vi "Log File Name for Mode.vi"(8 "error in":errorcluster, 9 "Mode":T1, 10 "base path":path) -> (0 "error out":errorcluster, 1 "for input Mode":path, 2 "for Create New":path, 3 "for Append":path, 5 "for Overwrite":path)   [LabVIEW 2021, in "Logging.lvlib"]
doc: "Take 'base path' and format it for presentation in the UI."
uses:
  Logging.lvlib
  Logging Mode.ctl
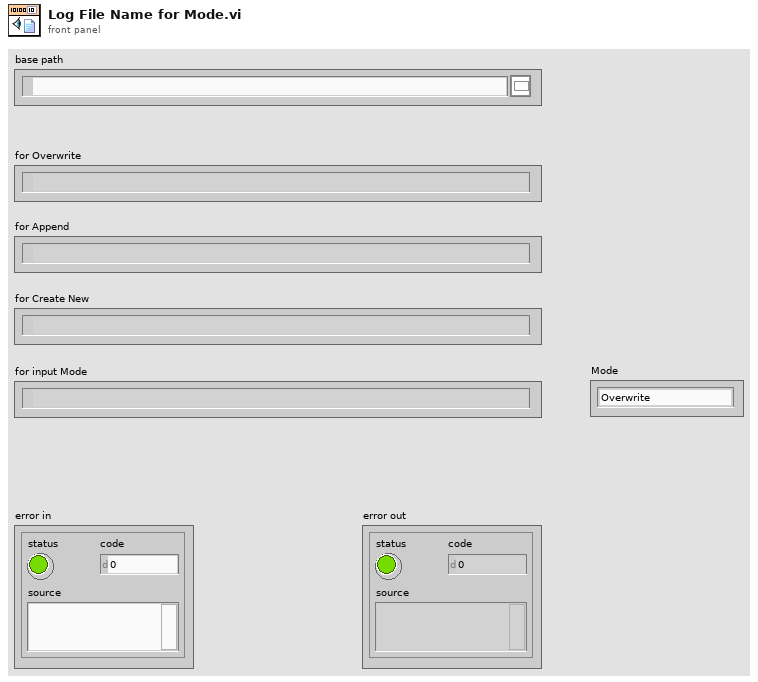
[diagram p1: front panel]
types:
  T1 = typedef "Logging.lvlib/Logging Mode.ctl" = enum16{"Overwrite", "Append", "Create New"}
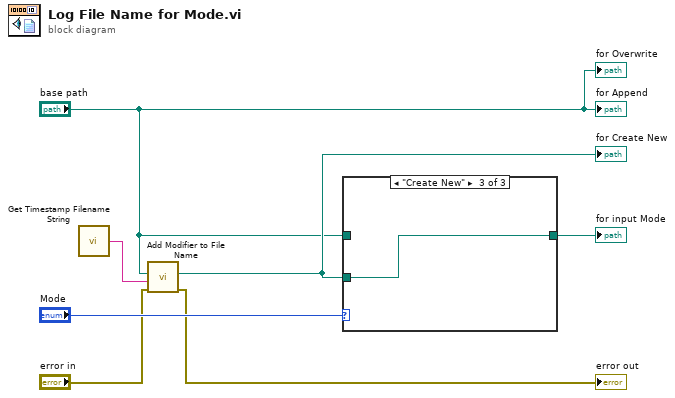
[diagram p0: block diagram]
diagram:
  n1 = call "Get Timestamp Filename String.vi"() -> ("time format string"=w7:string)
  n2 = call "Add Modifier to File Name.vi"("error in (no error)"="error in", "file name modifier"=w7, "base path"="base path") -> ("error out"=→"error out":errorcluster, "appended path"=w5:path)  [unwired: 7 in]
  "for Create New" <- w5
  n3 = case shown="\"Create New\"" "Mode" {
    tunnel: w5 -> [_ _ w10]
    tunnel: "base path" -> [w8 w9 _]
    tunnel: [w8 w9 w10] -> w3
    frame "Overwrite" {
    }
    frame "Append" {
    }
    frame "Create New" {
    }
  }
  "for input Mode" <- w3
  "for Overwrite" <- "base path"
  "for Append" <- "base path"
